vi "Rig_Editor.vi"(8 "error in (no error)":errorcluster={"status"=FALSE, "code"=0, "source"="\"\""}, 10 "resource metadata":string, 11 "RigDefinition":string) -> (0 "error out":errorcluster={"status"=FALSE, "code"=0, "source"="\"\""}, 2 "status ok":bool, 3 "Updated RigDefinition":string)   [LabVIEW 2026]
doc: "INTENT: Define rig resource and I/O capabilities. LOGIC: Show editable rig fields and parameter mappings; validate identifiers and protected limit permissions."
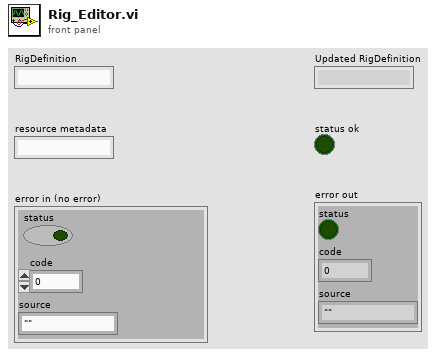
[diagram p1: front panel]
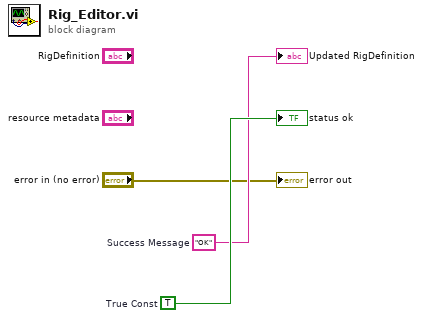
[diagram p0: block diagram]
diagram:
  w3 = TRUE  # True Const
  w2 = "OK"  # Success Message
  "Updated RigDefinition" <- w2
  "status ok" <- w3
  "error out" <- "error in (no error)"
